vi "Zad1.vi"() -> ()   [LabVIEW 2025]
uses:
  Zad1_enum.ctl
  d1481ebe-c914-40df-abee-77bc5e667ef0.vi
  <vilib>/Array/Sort 2D Array - Pop Stack.vi
  <vilib>/Array/Sort 2D Array - Push Stack.vi
  d1481ebe-c914-40df-abee-77bc5e667ef0.vi/269d4b3b-47f5-49e3-8884-44851e4dd9d5.vi
  d1481ebe-c914-40df-abee-77bc5e667ef0.vi/6d99389c-673d-4efb-bf33-19b32bcf4cf8.vi
panel:
  out "Output Array":dbl[][](array[numeric])
  in  "Input Array":dbl[][](array[numeric])
  in  "Sort by:":T1
  in  "Select row":dbl
  in  "Select column":dbl
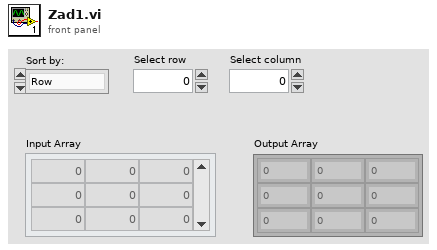
[diagram p1: front panel]
types:
  T1 = typedef "Zad1_enum.ctl" = enum16{"Row", "Column"}
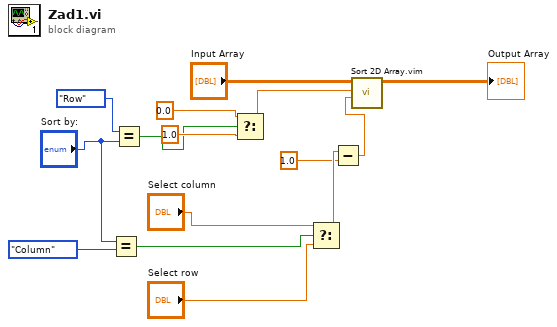
[diagram p0: block diagram]
diagram:
  n1 = Equal?(x="Sort by:", y=Zad1_enum."Column") -> (x = y?=w4:bool)
  n2 = Equal?(x=Zad1_enum."Row" ("y"), y="Sort by:") -> (x = y?=w10:bool)
  n3 = Select(t=0.0, s=w10, f=1.0) -> (s? t:f=w9:dbl)
  n4 = Select(t="Select column", s=w4, f="Select row") -> (s? t:f=w3:dbl)
  n5 = Subtract(x=w3, y=1.0) -> (x-y=w2:dbl)
  n6 = call "Sort 2D Array.vim"("index"=w2, "dimension to index (column)"=w9, "2D array"="Input Array") -> ("sorted 2D array"=→"Output Array":dbl[][])  [unwired: 7 in, 1 out]
